vi "Create Request.vi"(6 "notification? (F)":bool, 8 "error in (no error)":errorcluster, 9 "params":variant, 10 "method":string) -> (0 "error out":errorcluster, 2 "<JSON> Requests":string, 4 "IDs":string)   [LabVIEW 2019, in "JSON-RPC.lvlib"]
doc: "Format a Request object to send to a Server.\n\n<b>method</b> is a String containing the name of the method to be involked. Method names begining with \"rpc.\" are reserved for rpc-internal methods and extensions.\n\n<b>params</b> is a Structured value. The object will be formatted as follows:\n- Clusters will be flattened to json by-name\n- Arrays will be converted to json array\n- Elements (string, float, etc) will be converted to a 1 element json array\n\n<b>notification?</b> controls whether or not an id will be generated and sent. Requests without an id are treated as a notification and will not be responded to.\n\n<b>Note:</b> While the JSON-RPC spec supports batch Requests, this library currently does not have this feature.\n\nhttps://www.jsonrpc.org/specification"
uses:
  JSON-RPC.lvlib
  typedefs/Request--Cluster.ctl
  <vilib>/JDP Science/JSONtext/Make JSON Object.vi
  private/Create ID.vi
  private/Variant to JSONRPC params.vi
  <vilib>/Utility/MD5Checksum.llb/MD5Checksum string.vi
  <vilib>/JDP Science/JSONtext/support/Format JSON Object.vi
  <vilib>/JDP Science/JSONtext/support/Format JSON Array Text.vi
  <vilib>/JDP Science/JSONtext/JSONtext.lvlib
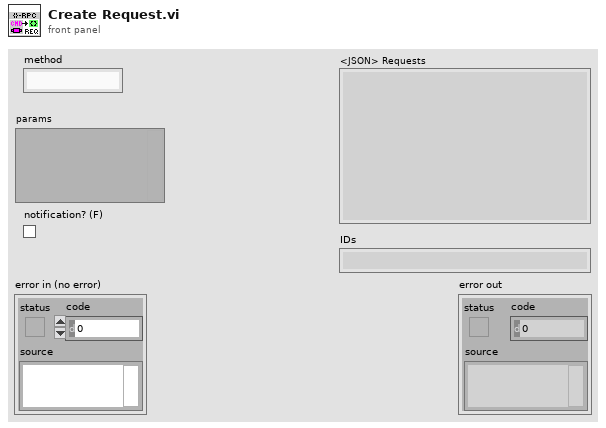
[diagram p1: front panel]
types:
  T1 = typedef "JSON-RPC.lvlib/Request--Cluster.ctl" = cluster{"jsonrpc":string, "method":string, "params":string, "id":string}
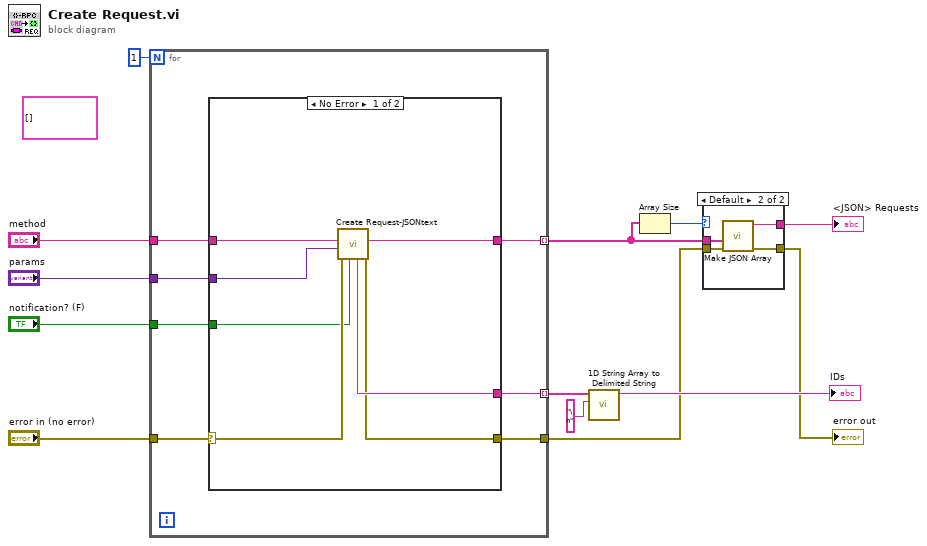
[diagram p0: block diagram]
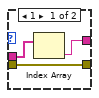
[diagram p2: hidden frame]
diagram:
  (unwired) T1[] [] ("Requests")
  n1 = for {
    N: 1 -> [_]
    tunnel: [w18] -> w9 mode=indexing
    tunnel: [w17] -> w6 mode=indexing
    tunnel: "error in (no error)" -> [w20]
    tunnel: [w19] -> w1
    tunnel: "notification? (F)" -> [w16]
    tunnel: "method" -> [w15]
    tunnel: "params" -> [w14]
    n2 = case shown="No Error" w20 {
      selector: w20 -> [w27 w28]
      tunnel: [w24 w28] -> w19
      tunnel: [w25 _] -> w18
      tunnel: [w26 _] -> w17
      tunnel: w16 -> [w23 _]
      tunnel: w15 -> [w22 _]
      tunnel: w14 -> [w21 _]
      frame No Error {
        n3 = call "Create Request-JSONtext.vi"("notification?"=w23, "error in (no error)"=w27, "params"=w21, "method"=w22) -> ("error out"=w24:errorcluster, "<JSON>"=w25:string, "id"=w26:string)  [unwired: 5 in]
      }
      frame Error {
      }
    }
  }
  n4 = call <vilib>:"1D String Array to Delimited String.vi"("delimiter"="\n", "string array"=w6) -> ("delimited string"=→"IDs":string)  [unwired: 9 in]
  n5 = Array Size(array=w9) -> (size(s)=w7:i32)
  n6 = case shown="Default" w7 {
    tunnel: [w30 w35] -> w12
    tunnel: w9 -> [w29 w34]
    tunnel: [w31 w33] -> w8
    tunnel: w1 -> [w31 w32]
    frame 1 {
      n7 = Index Array(array=w29) -> (element=w30:string)  [unwired: 1 in]
    }
    frame Default {
      n8 = call <vilib>:"Make JSON Array.vi"("error in (no error)"=w32, "JSON Elements"=w34) -> ("error out"=w33:errorcluster, "<JSON>"=w35:string)  [unwired: 8 in]
    }
  }
  "error out" <- w8
  "<JSON> Requests" <- w12
